vi "UI.vi"(8 "error in (no error)":errorcluster, 11 "View in":refnum<class "View.lvclass">) -> (0 "error out":errorcluster, 3 "View out":refnum<class "View.lvclass">)   [LabVIEW 2024, in "View.lvclass"]
uses:
  View.lvclass
  UIRefs.ctl
  View.lvclass/View.ctl
  Viewmodel/Viewmodel.lvclass
  C:/Users/N Tan/Documents/1-Reuse Modules/ReactiveState/ChangeNotifier/ChangeNotifier.lvclass
  ChangeNotifier/ChangeNotifier.lvclass
panel:
  in  "Decrement":bool
  in  "Increment":bool
  out "Counter":i32
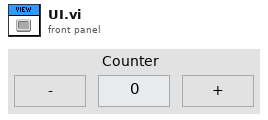
[diagram p1: front panel]
types:
  T1 = typedef "View.lvclass/UIRefs.ctl" = cluster{"Counter":refnum<vi>, "Increment":refnum<vi>, "Decrement":refnum<vi>}
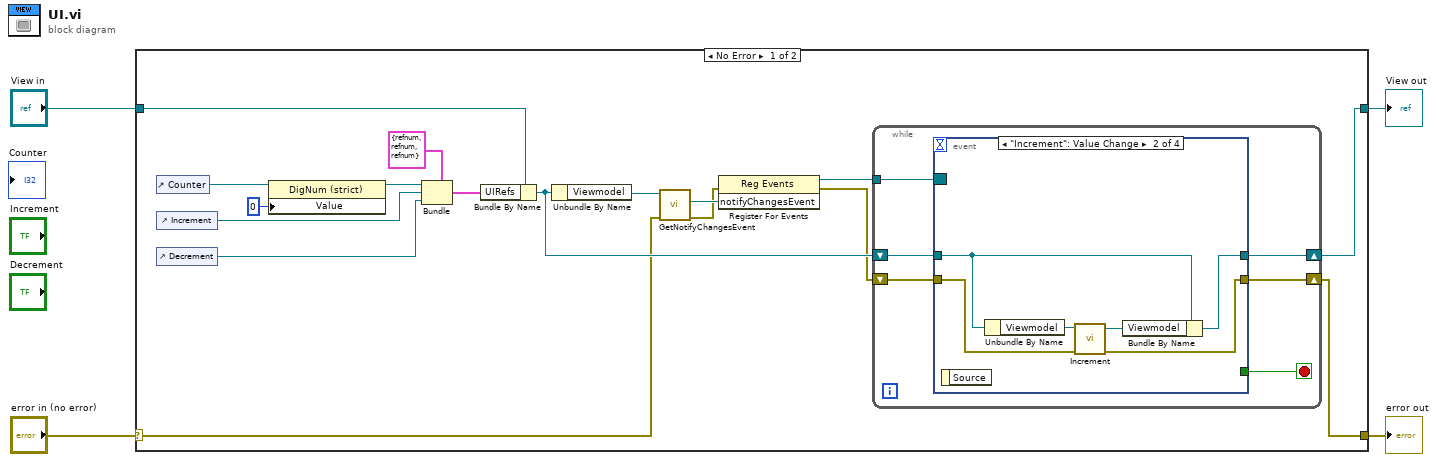
[diagram p0: block diagram]
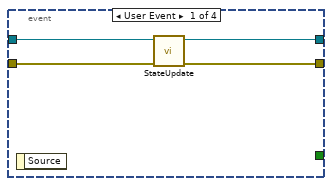
[diagram p2: hidden frame]
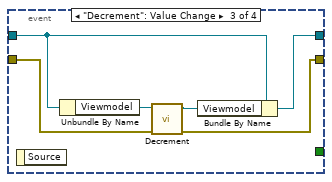
[diagram p3: hidden frame]
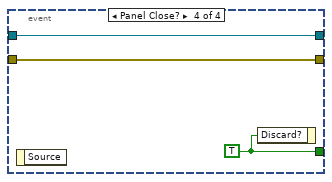
[diagram p4: hidden frame]
diagram:
  n1 = case shown="No Error" "error in (no error)" {
    selector: "error in (no error)" -> [w10 w48]
    tunnel: [w13 w48] -> w3
    tunnel: [w12 w47] -> w1
    tunnel: "View in" -> [w18 w47]
    frame No Error {
      n2 = control-ref of="Counter"() -> (w7:refnum<vi>)
      n3 = control-ref of="Increment"() -> (w21:refnum<vi>)
      n4 = control-ref of="Decrement"() -> (w20:refnum<vi>)
      n5 = property class="DigNum (strict)"(reference=w7, "Value"=0) -> (reference out=w6:refnum<vi>)  [unwired: 1 in, 1 out]
      n6 = Bundle(cluster=T1 {"Counter"=refnum, "Increment"=refnum, "Decrement"=refnum} ("output cluster"), "Counter"=w6, "Increment"=w21, "Decrement"=w20) -> (w17:T1)
      n7 = Bundle By Name(cluster=w18, "UIRefs"=w17) -> (w15:refnum<class "View.lvclass">)
      n8 = Unbundle By Name(w15) -> ("Viewmodel"=w11:refnum<class "Viewmodel.lvclass">)
      n9 = call "GetNotifyChangesEvent.vi"("error in (no error)"=w10, "ChangeNotifier in"=w11) -> ("error out"=w8:errorcluster, "notifyChangesEvent"=w9:refnum<user-event>)  [unwired: 7 in, 1 out]
      n10 = register-events(error in=w8, w9) -> (reference out=w16:refnum<event-registration>, error out=w14:errorcluster)  [unwired: 1 in]
      n11 = while {
        tunnel: w16 -> [w26]
        shift-right: [w24] -> w12
        shift-left: w15 -> [w25]
        shift-right: [w23] -> w13
        shift-left: w14 -> [w22]
        stop <- w27 stop-if-true
        n12 = event shown="[1] \"Increment\": Value Change" {
          selector: w26 -> [_ _ _ _]
          dyn-events: _ -> [_ _ _ _]
          timeout: _ -> [_ _ _ _]
          tunnel: [_ _ _ w46] -> w27
          tunnel: w25 -> [w31 w34 w43 w45]
          tunnel: [w30 w33 w42 w45] -> w24
          tunnel: [w29 w32 w40 w44] -> w23
          tunnel: w22 -> [w28 w37 w41 w44]
          event User Event {
            n13 = event-data() -> ()  [unwired: 1 in, 1 out]
            n14 = call "StateUpdate.vi"("error in (no error)"=w28, "View in"=w31) -> ("error out"=w29:errorcluster, "View out"=w30:refnum<class "View.lvclass">)  [unwired: 8 in]
          }
          event "Increment": Value Change {
            n15 = event-data() -> ()  [unwired: 1 in, 1 out]
            n16 = Unbundle By Name(w34) -> ("Viewmodel"=w36:refnum<class "Viewmodel.lvclass">)
            n17 = call "Increment.vi"("error in (no error)"=w37, "Viewmodel in"=w36) -> ("error out"=w32:errorcluster, "Viewmodel out"=w35:refnum<class "Viewmodel.lvclass">)  [unwired: 8 in]
            n18 = Bundle By Name(cluster=w34, "Viewmodel"=w35) -> (w33:refnum<class "View.lvclass">)
          }
          event "Decrement": Value Change {
            n19 = event-data() -> ()  [unwired: 1 in, 1 out]
            n20 = Unbundle By Name(w43) -> ("Viewmodel"=w38:refnum<class "Viewmodel.lvclass">)
            n21 = call "Decrement.vi"("error in (no error)"=w41, "Viewmodel in"=w38) -> ("error out"=w40:errorcluster, "Viewmodel out"=w39:refnum<class "Viewmodel.lvclass">)  [unwired: 8 in]
            n22 = Bundle By Name(cluster=w43, "Viewmodel"=w39) -> (w42:refnum<class "View.lvclass">)
          }
          event Panel Close? {
            w46 = TRUE
            n23 = event-data() -> ()  [unwired: 1 in, 1 out]
            n24 = event-data("Discard?"=w46) -> ()  [unwired: 1 in, 1 out]
          }
        }
      }
    }
    frame Error {
    }
  }
  "error out" <- w3
  "View out" <- w1
